vi "PR_CTICA3_PARTE_B.vi"() -> ()   [LabVIEW 2026]
panel:
  in  "Valor":dbl
  in  "Array":dbl[][](array[numeric])
  in  "Columna":dbl
  in  "Fila":dbl
  out "Indicadores":dbl[][](array[numeric])
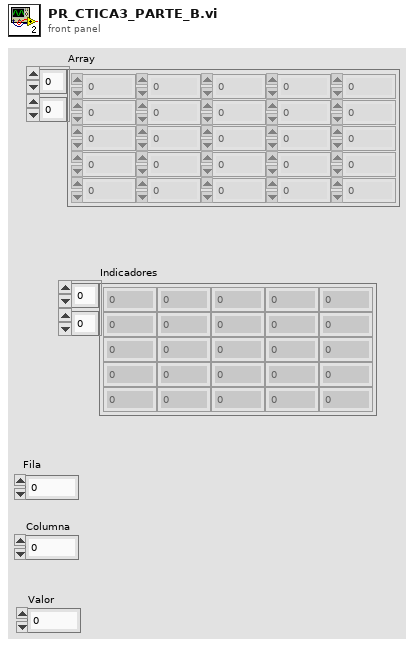
[diagram p1: front panel]
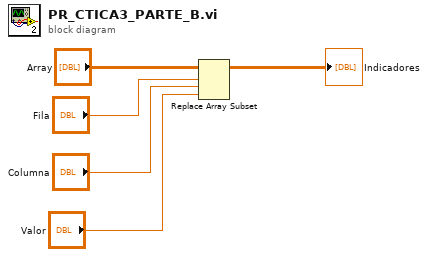
[diagram p0: block diagram]
diagram:
  n1 = Replace Array Subset(array="Array", new element="Valor", index (row)="Fila", index (col)="Columna") -> (→"Indicadores":dbl[][])
